vi "Water side capacity.vi"(10 "Pressure and Flow meter in":T2, 11 "RTD Data ID & OD":T1={"ID_Noz_DBT"=30.10343849658966, "ID_UUT_Inlet_WBT"=34.19517338275909, "ID_UUT_Inlet_DBT"=34.22250419855118, "ID_UUT_Outlet DBT"=32.61692941188812, "ID_UUT_Outlet WBT"=32.61692941188812, "ID EWT"=32.61692941188812, "ID LWT"=32.61692941188812, "OD_UUT_Inlet_WBT"=33.95874559879303, "OD_UUT_Inlet_DBT"=35.07717490196227, "OD_UUT_Outlet_DBT "=33.95874559879303} {"OD_UUT_Outlet_DBT" format="%0.2f"; "OD_UUT_Inlet_DBT" format="%0.2f"; "OD_UUT_Inlet_WBT" format="%0.2f"; "ID LWT" format="%0.2f"; "ID EWT" format="%0.2f"; "ID_UUT_Outlet WBT" format="%0.2f"; "ID_UUT_Outlet DBT" format="%0.2f"; "ID_UUT_Inlet_DBT" format="%0.2f"; "ID_UUT_Inlet_WBT" format="%0.2f"; "ID_Noz_DBT" format="%0.2f"}) -> (1 "FCU EWT":dbl, 2 "FCU WFR 2":dbl, 3 "WCC":dbl, 4 "FCU LWT":dbl, 5 "FCU Water PD 2":dbl)   [LabVIEW 2025]
uses:
  Global Variables/General Glob.vi
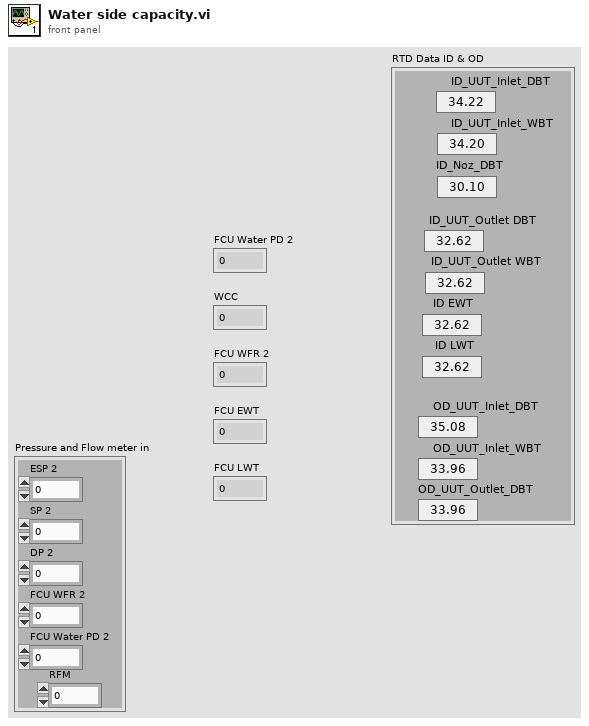
[diagram p1: front panel]
types:
  T1 = cluster{"ID_Noz_DBT":dbl, "ID_UUT_Inlet_WBT":dbl, "ID_UUT_Inlet_DBT":dbl, "ID_UUT_Outlet DBT":dbl, "ID_UUT_Outlet WBT":dbl, "ID EWT":dbl, "ID LWT":dbl, "OD_UUT_Inlet_WBT":dbl, "OD_UUT_Inlet_DBT":dbl, "OD_UUT_Outlet_DBT ":dbl}
  T2 = cluster{"ESP 2":dbl, "SP 2":dbl, "DP 2":dbl, "FCU WFR 2":dbl, "FCU Water PD 2":dbl, "RFM":dbl}
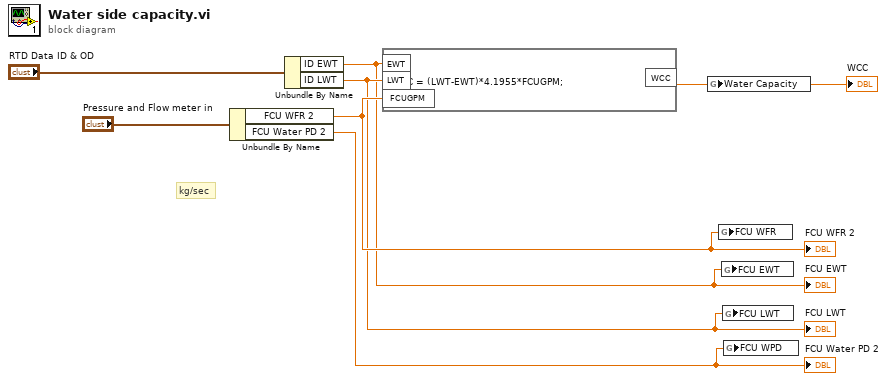
[diagram p0: block diagram]
diagram:
  # "kg/sec"
  n1 = Unbundle By Name("Pressure and Flow meter in") -> ("FCU WFR 2"=w5:dbl, "FCU Water PD 2"=w3:dbl)
  "FCU Water PD 2" <- w3
  "FCU WFR 2" <- w5
  n2 = Unbundle By Name("RTD Data ID & OD") -> ("ID EWT"=w1:dbl, "ID LWT"=w4:dbl)
  "FCU LWT" <- w4
  "FCU EWT" <- w1
  n3 = formula code="WCC = (LWT-EWT)*4.1955*FCUGPM;"("EWT"=w1, "LWT"=w4, "FCUGPM"=w5) -> ("WCC"=w7:dbl)
  "WCC" <- w7
  n4 = global write "General Glob.vi" "Water Capacity"(w7) -> ()
  n5 = global write "General Glob.vi" "FCU WFR"(w5) -> ()
  n6 = global write "General Glob.vi" "FCU EWT"(w1) -> ()
  n7 = global write "General Glob.vi" "FCU LWT"(w4) -> ()
  n8 = global write "General Glob.vi" "FCU WPD"(w3) -> ()
